vi "子VI-Openx.vi"(0 "超时":u32, 1 "地址":string) -> (2 "描述":string, 3 "会话":u32=4294967295, 4 "返回值":i32)   [LabVIEW 2011]
panel:
  out "error out":errorcluster caption="错误输出"
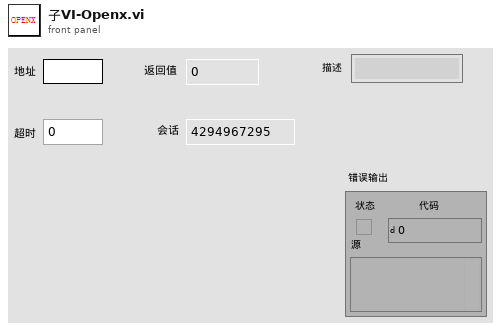
[diagram p1: front panel]
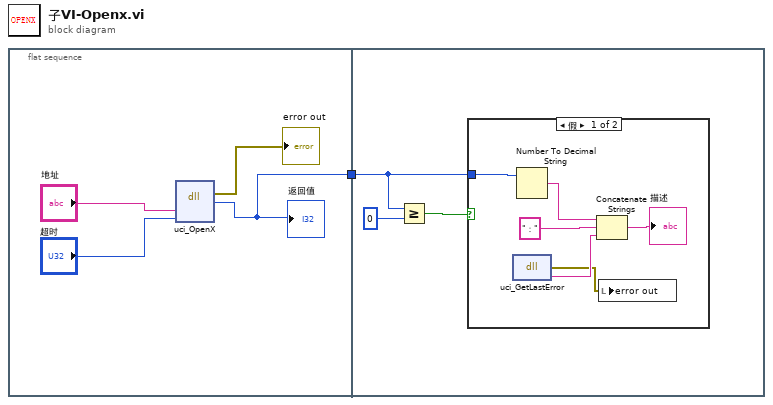
[diagram p0: block diagram]
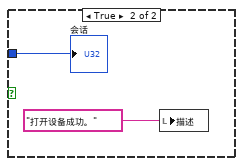
[diagram p2: hidden frame]
diagram:
  n1 = flat-sequence {
    tunnel: [w2] -> w1
    tunnel: w1 -> [w6]
    frame #0 {
      n2 = dll-call lib="PTH1Eabs E调试程序\nLabView程序UCI示例程序ASCIIuci.dll" fn="uci_OpenX"("addr"="地址", "timeout"="超时") -> (error out=→"error out":errorcluster, "返回类型"=w2:i32)  [unwired: 5 in, 1 out]
      "返回值" <- w2
    }
    frame #1 {
      n3 = Greater Or Equal?(x=w6, y=0) -> (x >= y?=w7:bool)
      n4 = case shown="假" w7 {
        tunnel: w6 -> [w14 w16]
        frame False {
          n5 = dll-call lib="PTH1Eabs E调试程序\nLabView程序UCI示例程序ASCIIuci.dll" fn="uci_GetLastError"() -> (error out=w9:errorcluster, "返回类型"=w11:string)  [unwired: 3 in, 1 out]
          n6 = Number To Decimal String(number=w14) -> (decimal integer string=w13:string)  [unwired: 1 in]
          n7 = Concatenate Strings(w13, "：", w11) -> (→"描述":string)
          n8 = local write "error out"(w9) -> ()
        }
        frame True {
          n9 = local write "描述"("打开设备成功。") -> ()
          "会话" <- w16
        }
      }
    }
  }
